vi "Read User Data.vi"(8 "error in (no error)":errorcluster, 11 "User Data Path":path) -> (0 "error out":errorcluster, 3 "data out":T1)   [LabVIEW 2018]
doc: "Reads the user data stored in the configuration file specified by <b>User Data Path</b>. Opens the configuration file, retrieves its contents and returns the data through the data out output. Closes the file reference and propagates any errors through the error cluster."
uses:
  <vilib>/TABOADA/Config Files Management/Config Files Management/config data--cluster.ctl
  <vilib>/TABOADA/Config Files Management/Config Files Management/Config Files Management.lvlib
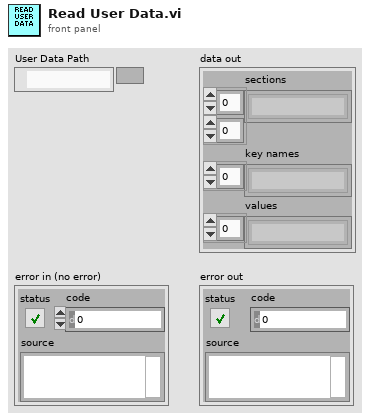
[diagram p1: front panel]
types:
  T1 = typedef "Config Files Management.lvlib/config data--cluster.ctl" = cluster{"sections":string[][], "key names":string[], "values":string[]}
  T2 = typedef "NI_LVConfig.lvlib/Config Data RefNum.ctl" = refnum<k1>
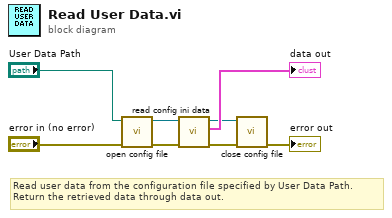
[diagram p0: block diagram]
diagram:
  # "Read user data from the configuration file specified by User Data Path.\nReturn the retrieved data through data out."
  n1 = call <vilib>:"open config file.vi"("error in (no error)"="error in (no error)", "configuration file path"="User Data Path") -> ("error out"=w2:errorcluster, "Refnum out"=w3:T2)  [unwired: 7 in, 1 out]
  n2 = call <vilib>:"read config ini data.vi"("error in (no error)"=w2, "Refnum in"=w3) -> ("error out"=w4:errorcluster, "data out"=→"data out":T1, "Refnum out"=w5:T2)  [unwired: 7 in]
  n3 = call <vilib>:"close config file.vi"("error in (no error)"=w4, "Refnum in"=w5) -> ("error out"=→"error out":errorcluster)  [unwired: 9 in]
